vi "query Sweep Point.vi"(8 "error in (no error)":errorcluster, 11 "Keysight 9020A in":refnum<class "Keysight 9020A.lvclass">) -> (0 "error out":errorcluster, 2 "Sweep Point":u32, 3 "Keysight 9020A out":refnum<class "Keysight 9020A.lvclass">)   [LabVIEW 2023, in "Spectrum Analyzer.lvlib" / "Keysight 9020A.lvclass"]
uses:
  Keysight 9020A.lvclass
  Keysight 9020A.lvclass/Keysight 9020A.ctl
  Spectrum Analyzer.lvlib
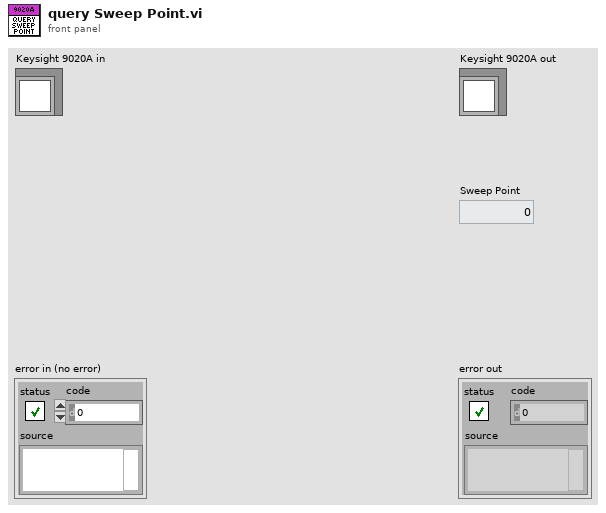
[diagram p1: front panel]
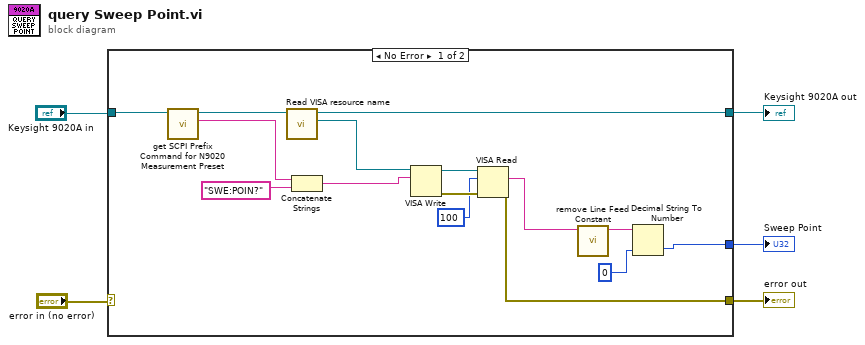
[diagram p0: block diagram]
diagram:
  n1 = case shown="No Error" "error in (no error)" {
    selector: "error in (no error)" -> [_ w21]
    tunnel: "Keysight 9020A in" -> [w10 w22]
    tunnel: [w20 w22] -> w3
    tunnel: [w13 w21] -> w2
    tunnel: [w12 _] -> w1
    frame No Error {
      n2 = call "get SCPI Prefix Command for N9020 Measurement Preset.vi"("Keysight 9020A in"=w10) -> ("SCPI Prefix Command"=w7:string, "Keysight 9020A out"=w9:refnum<class "Keysight 9020A.lvclass">)  [unwired: 8 in, 1 out]
      n3 = call "Read VISA resource name.vi"("Keysight 9020A in"=w9) -> ("VISA resource name"=w15:refnum<visa-resource-name>, "Keysight 9020A out"=w20:refnum<class "Keysight 9020A.lvclass">)  [unwired: 8 in, 1 out]
      n4 = Concatenate Strings(w7, "SWE:POIN?" ("write buffer")) -> (w6:string)
      n5 = VISA Write(VISA resource name=w15, write buffer=w6) -> (VISA resource name out=w19:refnum<visa-resource-name>, error out=w18:errorcluster)  [unwired: 1 in, 1 out]
      n6 = VISA Read(VISA resource name=w19, byte count=u32 100, error in (no error)=w18) -> (read buffer=w16:string, error out=w13:errorcluster)  [unwired: 2 out]
      n7 = call "remove Line Feed Constant.vi"("Input String"=w16) -> ("Line Feed Removed String"=w14:string)  [unwired: 10 in]
      n8 = Decimal String To Number(string=w14, default (0L)=u32 0) -> (number=w12:u32)  [unwired: 1 in, 1 out]
    }
    frame Error {
    }
  }
  "error out" <- w2
  "Keysight 9020A out" <- w3
  "Sweep Point" <- w1
